vi "Configure Module.vi"(8 "error in (no error)":errorcluster, 10 "IOV ref in":variant, 11 "9235 in":refnum<class "9235.lvclass">) -> (0 "error out":errorcluster, 2 "IOV ref out":variant, 3 "9235 out":refnum<class "9235.lvclass">)   [LabVIEW 2020, in "Modules.lvlib" / "9235.lvclass"]
uses:
  9235.lvclass
  <resource>/objmgr/cRIO.rc
  RSI Module/RSI Module.lvclass
  C:/Users/nitest/Desktop/Git 2020/niveristand-scan-engine-module-libraries/Source/RSI Module/RSI Module.lvclass
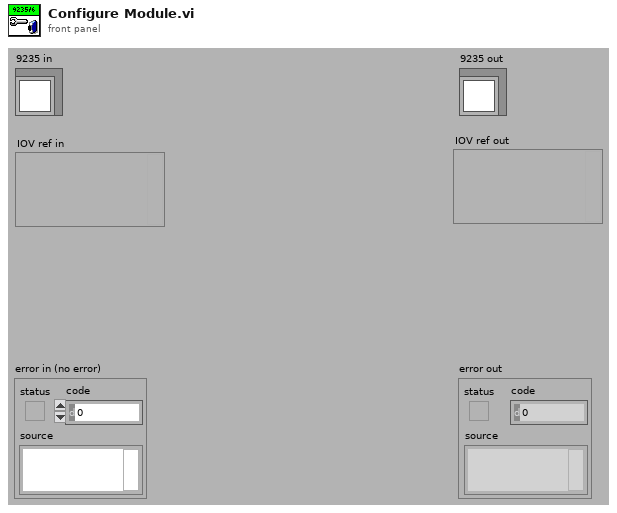
[diagram p1: front panel]
types:
  T1 = typedef "Modules.lvlib/RSI Module.lvclass/Module Models.ctl" = enum16{"Empty", "NI 9201", "NI 9203", "NI 9205", "NI 9206", "NI 9207", "NI 9208", "NI 9209", "NI 9210", "NI 9211", "NI 9212", "NI 9213", "NI 9214", "NI 9215", "NI 9216", "NI 9217", "NI 9219", "NI 9220", "NI 9221", "NI 9222", "NI 9223", "NI 9224", "NI 9225", "NI 9226", "NI 9227", "NI 9228", "NI 9229", "NI 9233", "NI 9234", "NI 9235", "NI 9236", "NI 9237", "NI 9239", "NI 9242", "NI 9244", "NI 9253", "NI 9263", "NI 9264", "NI 9265", "NI 9266", "NI 9269", "NI 9344", "NI 9350", "NI 9375", "NI 9401", "NI 9402", "NI 9403", "NI 9411", "NI 9421", "NI 9422", "NI 9423", "NI 9425", "NI 9426", "NI 9435", "NI 9436", "NI 9437", "NI 9472", "NI 9474", "NI 9475", "NI 9476", "NI 9477", "NI 9478", "NI 9481", "NI 9482", "NI 9485"}
  T2 = typedef "Modules.lvlib/9235.lvclass/Data rate.ctl" = u32
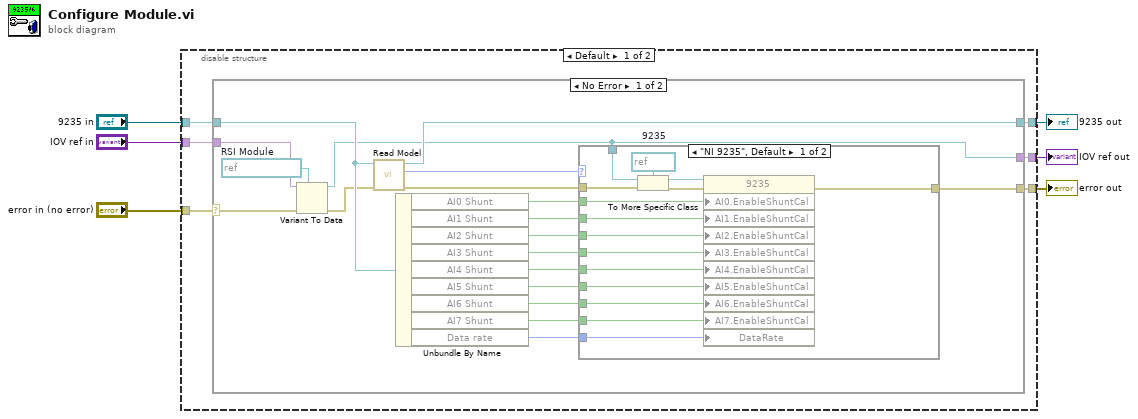
[diagram p0: block diagram]
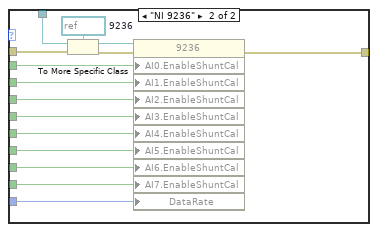
[diagram p2: hidden frame]
diagram:
  n1 = disable-structure shown="Default" {
    disable-tunnel: "error in (no error)" -> [w12 w67]
    disable-tunnel: [w11 w67] -> w5
    disable-tunnel: "9235 in" -> [w10 w65]
    disable-tunnel: [w9 w65] -> w3
    disable-tunnel: "IOV ref in" -> [w8 w66]
    disable-tunnel: [w7 w66] -> w1
    frame condition #0 {
      n2 = case shown="No Error" w12 {
        selector: w12 -> [w21 w64]
        tunnel: [w22 w64] -> w11
        tunnel: [w18 w63] -> w9
        tunnel: w10 -> [w19 w63]
        tunnel: w8 -> [w15 w62]
        tunnel: [w14 w62] -> w7
        frame No Error {
          w13 = refnum<k21> refnum  # RSI Module
          n3 = Variant To Data(error in=w21, type=w13, Variant=w15) -> (data=w14:refnum<k21>, error out=w16:errorcluster)
          n4 = call "Read Model.vi"("error in (no error)"=w16, "RSI Module in"=w19) -> ("error out"=w20:errorcluster, "Model"=w17:T1, "RSI Module out"=w18:refnum<class "9235.lvclass">)  [unwired: 7 in]
          n5 = Unbundle By Name(w19) -> ("AI0 Shunt"=w31:bool, "AI1 Shunt"=w30:bool, "AI2 Shunt"=w29:bool, "AI3 Shunt"=w28:bool, "AI4 Shunt"=w27:bool, "AI5 Shunt"=w26:bool, "AI6 Shunt"=w25:bool, "AI7 Shunt"=w24:bool, "Data rate"=w23:T2)
          n6 = case shown="\"NI 9235\", Default" w17 {
            tunnel: w14 -> [w44 w59]
            tunnel: w31 -> [w42 w57]
            tunnel: w30 -> [w41 w56]
            tunnel: w29 -> [w40 w55]
            tunnel: w28 -> [w39 w54]
            tunnel: w27 -> [w38 w53]
            tunnel: w26 -> [w37 w52]
            tunnel: w25 -> [w36 w51]
            tunnel: w24 -> [w35 w50]
            tunnel: w23 -> [w34 w49]
            tunnel: [w33 w48] -> w22
            tunnel: w20 -> [w32 w47]
            frame "NI 9235", Default {
              w46 = refnum<k21> refnum  # 9235
              n7 = To More Specific Class(target class=w46, reference=w44, error in=w32) -> (specific class reference=w43:refnum<k21>, error out=w45:errorcluster)
              n8 = property class="9235"(reference=w43, error in=w45, "AI0.EnableShuntCal"=w42, "AI1.EnableShuntCal"=w41, "AI2.EnableShuntCal"=w40, "AI3.EnableShuntCal"=w39, "AI4.EnableShuntCal"=w38, "AI5.EnableShuntCal"=w37, "AI6.EnableShuntCal"=w36, "AI7.EnableShuntCal"=w35, "DataRate"=w34) -> (error out=w33:errorcluster)  [unwired: 1 out]
            }
            frame "NI 9236" {
              w61 = refnum<k21> refnum  # 9236
              n9 = To More Specific Class(target class=w61, reference=w59, error in=w47) -> (specific class reference=w58:refnum<k21>, error out=w60:errorcluster)
              n10 = property class="9236"(reference=w58, error in=w60, "AI0.EnableShuntCal"=w57, "AI1.EnableShuntCal"=w56, "AI2.EnableShuntCal"=w55, "AI3.EnableShuntCal"=w54, "AI4.EnableShuntCal"=w53, "AI5.EnableShuntCal"=w52, "AI6.EnableShuntCal"=w51, "AI7.EnableShuntCal"=w50, "DataRate"=w49) -> (error out=w48:errorcluster)  [unwired: 1 out]
            }
          }
        }
        frame Error {
        }
      }
    }
    frame condition #1 (active) {
    }
  }
  "error out" <- w5
  "9235 out" <- w3
  "IOV ref out" <- w1
